vi "Delete Session State.vi"(8 "error in (no error)":errorcluster, 11 "Client ID":string) -> (0 "error out":errorcluster, 1 "Found?":bool)   [LabVIEW 2013, in "MQTT Server.lvlib" / "StoredSessions.lvclass"]
uses:
  StoredSessions.lvclass
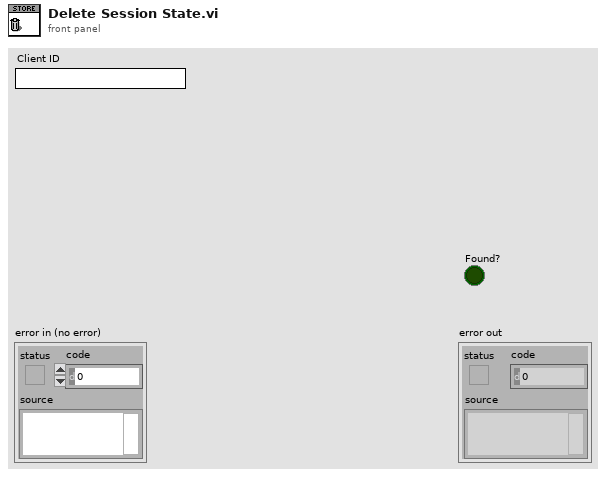
[diagram p1: front panel]
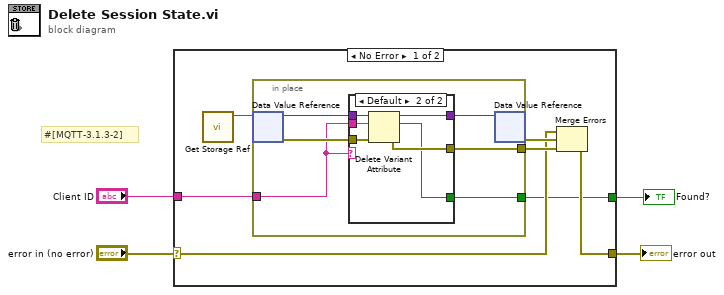
[diagram p0: block diagram]
diagram:
  # "#[MQTT-3.1.3-2]"
  n1 = case shown="No Error" "error in (no error)" {
    selector: "error in (no error)" -> [w7 w26]
    tunnel: [w6 w26] -> w3
    tunnel: "Client ID" -> [w10 _]
    tunnel: [w5 _] -> w1
    frame No Error {
      n2 = call "Get Storage Ref.vi"() -> ("Storage"=w11:refnum<data-value>)  [unwired: 11 in]
      n3 = in-place {
        in-place-border: w10 -> [w12]
        in-place-border: [w16] -> w9
        in-place-border: [w13] -> w5
        n4 = in-place-dvr #1(w11) -> (w14:variant, w15:errorcluster)
        n5 = case shown="Default" w12 {
          tunnel: [w19 w25] -> w17
          tunnel: [w18 w24] -> w16
          tunnel: w15 -> [w18 w23]
          tunnel: w14 -> [w19 w22]
          tunnel: w12 -> [_ w21]
          tunnel: [_ w20] -> w13
          frame "" {
          }
          frame Default {
            n6 = Delete Variant Attribute(4:w23, 6:w21, 7:w22) -> (0:w24:errorcluster, 2:w20:bool, 3:w25:variant)
          }
        }
        n7 = in-place-dvr #1(w17) -> (w8:errorcluster)  [unwired: 1 out]
      }
      n8 = Merge Errors(w7, w8, w9) -> (w6:errorcluster)
    }
    frame Error {
    }
  }
  "error out" <- w3
  "Found?" <- w1
